vi "Write_Raw.vi"(7 "n frames":u32, 8 "error in (no error)":errorcluster, 9 "length":i32, 10 "bytes in":u8[](array[numeric]), 11 "channel in":refnum<class "CANsub_DirectChannel.lvclass">) -> (0 "error out":errorcluster, 2 "bytes out":u8[](array[numeric]), 3 "channel out":refnum<class "CANsub_DirectChannel.lvclass">)   [LabVIEW 2021, in "CANsub_API.lvlib" / "CANsub_DirectChannel.lvclass"]
doc: "Sends a buffer of WebSocket frames that the caller prepared (for example with C_CIF_Encode_RT) with one TCP Write. length is the number of valid bytes in bytes in. n frames is the number of CAN frames in the buffer; it is added to frames written in the status. Loop-safe: no allocation in this class, bounded time (TCP Write timeout 1 s)."
uses:
  CANsub_DirectChannel.lvclass
  CANsub_DirectChannel.lvclass/CANsub_DirectChannel.ctl
  CANsub_API.lvlib
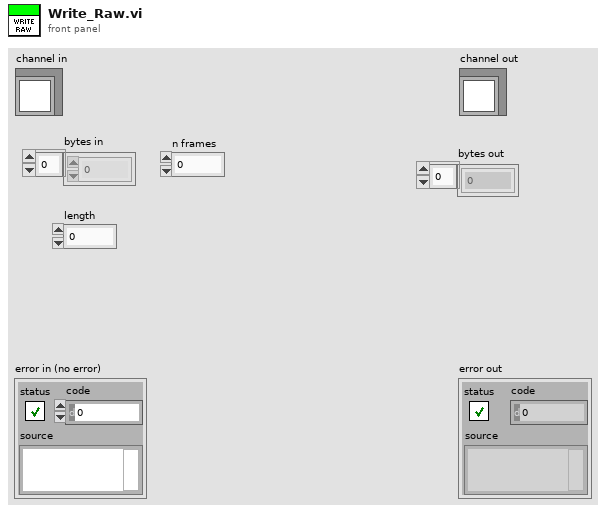
[diagram p1: front panel]
types:
  T1 = typedef "CANsub_API.lvlib/CANsub_Status.ctl" = cluster{"state":T2, "frames read":u32, "frames written":u32, "crc errors":u32, "decode errors":i32, "pings":u32, "FIFO overflows":u32, "reopens":u32, "nodelay":i32, "api version":string, "lib version":u32, "bit timing":T3, "last error":errorcluster}
  T2 = typedef "CANsub_API.lvlib/CANsub_State.ctl" = enum16{"Closed", "Open", "Lost"}
  T3 = typedef "CANsub_Common.lvlib/Bit_Timing.ctl" = cluster{"brp":u16, "seg1":u16, "seg2":u16, "sjw":u16, "data brp":u16, "data seg1":u16, "data seg2":u16, "data sjw":u16}
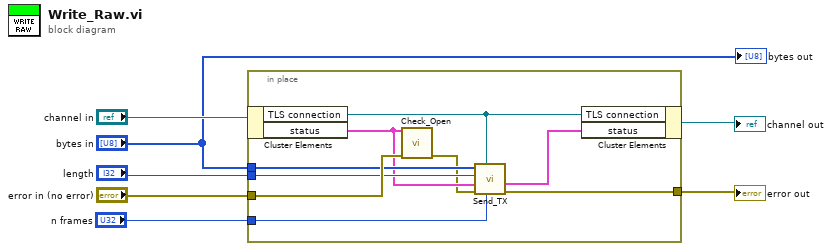
[diagram p0: block diagram]
diagram:
  n1 = in-place {
    in-place-border: [w15] -> w6
    in-place-border: "error in (no error)" -> [w14]
    in-place-border: "bytes in" -> [w13]
    in-place-border: "length" -> [w12]
    in-place-border: "n frames" -> [w8]
    n2 = in-place-cluster #1("channel in") -> ("TLS connection"=w11:refnum<k5>, "status"=w10:T1)
    n3 = call "Check_Open.vi"("error in (no error)"=w14, "status"=w10) -> ("error out"=w9:errorcluster)  [unwired: 9 in]
    n4 = call "Send_TX.vi"("frames (1)"=w8, "TLS connection"=w11, "error in (no error)"=w9, "status in"=w10, "length"=w12, "tx"=w13) -> ("error out"=w15:errorcluster, "status out"=w16:T1)  [unwired: 4 in]
    n5 = in-place-cluster #1("TLS connection"=w11, "status"=w16) -> (→"channel out":refnum<class "CANsub_DirectChannel.lvclass">)
  }
  "error out" <- w6
  "bytes out" <- "bytes in"
